vi "request OBW Measurement.vi"(8 "error in (no error)":errorcluster, 10 "Query Mode":T1, 11 "Keysight 9020A in":refnum<class "Keysight 9020A.lvclass">) -> (0 "error out":errorcluster, 2 "OBW Measurement Result Array":dbl[](array[numeric]), 3 "Keysight 9020A out":refnum<class "Keysight 9020A.lvclass">)   [LabVIEW 2023, in "Spectrum Analyzer.lvlib" / "Keysight 9020A.lvclass"]
uses:
  Keysight 9020A.lvclass
  TYPE DEFINITION/TYPE query Data Processing Type.ctl
  Keysight 9020A.lvclass/Keysight 9020A.ctl
  Spectrum Analyzer.lvlib
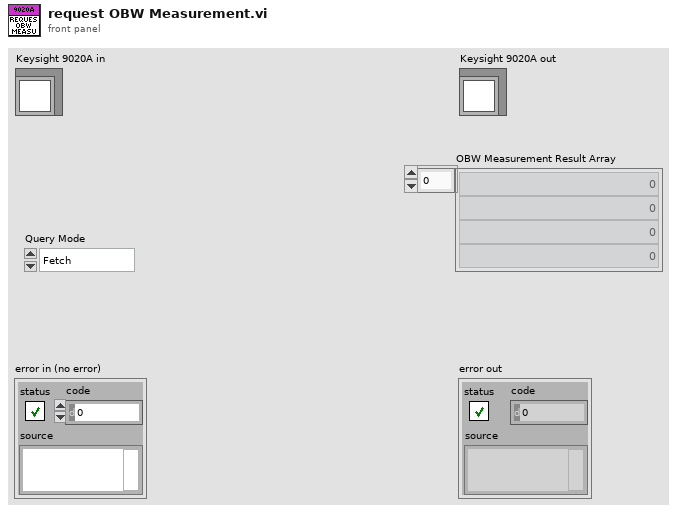
[diagram p1: front panel]
types:
  T1 = typedef "Spectrum Analyzer.lvlib/TYPE query Data Processing Type.ctl" = enum16{"Fetch", "Measure", "Read"}
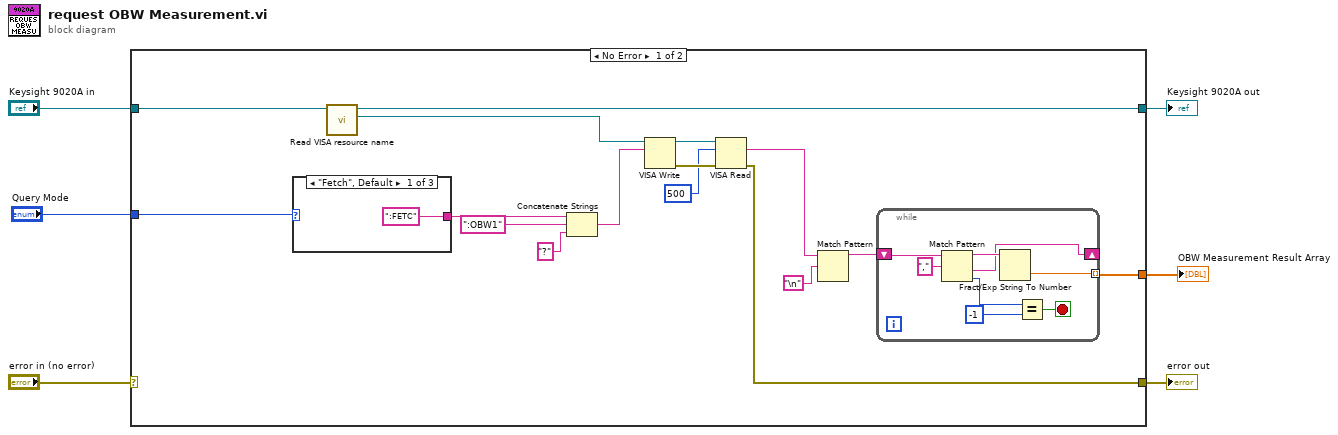
[diagram p0: block diagram]
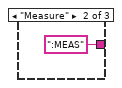
[diagram p2: hidden frame]
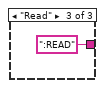
[diagram p3: hidden frame]
diagram:
  n1 = case shown="No Error" "error in (no error)" {
    selector: "error in (no error)" -> [_ w35]
    tunnel: [w8 w35] -> w5
    tunnel: [w18 w34] -> w3
    tunnel: "Keysight 9020A in" -> [w7 w34]
    tunnel: "Query Mode" -> [w19 _]
    tunnel: [w9 _] -> w1
    frame No Error {
      n2 = case shown="\"Fetch\", Default" w19 {
        tunnel: [":FETC" ":MEAS" ":READ"] -> w22
        frame "Fetch", Default {
        }
        frame "Measure" {
        }
        frame "Read" {
        }
      }
      n3 = call "Read VISA resource name.vi"("Keysight 9020A in"=w7) -> ("VISA resource name"=w11:refnum<visa-resource-name>, "Keysight 9020A out"=w18:refnum<class "Keysight 9020A.lvclass">)  [unwired: 8 in, 1 out]
      n4 = Concatenate Strings(w22, ":OBW1" ("string"), "?" ("string")) -> (w10:string)
      n5 = VISA Write(VISA resource name=w11, write buffer=w10) -> (VISA resource name out=w16:refnum<visa-resource-name>, error out=w17:errorcluster)  [unwired: 1 in, 1 out]
      n6 = VISA Read(VISA resource name=w16, byte count=u32 500, error in (no error)=w17) -> (read buffer=w14:string, error out=w8:errorcluster)  [unwired: 2 out]
      n7 = Match Pattern(string=w14, regular expression="\n") -> (before substring=w12:string)  [unwired: 1 in, 3 out]
      n8 = while {
        shift-right: [w26] -> _
        shift-left: w12 -> [w30]
        tunnel: [w27] -> w9 mode=indexing
        stop <- w23 stop-if-true
        n9 = Match Pattern(string=w30, regular expression=",") -> (before substring=w28:string, after substring=w26:string, offset past match=w25:i32)  [unwired: 1 in, 1 out]
        n10 = Fract/Exp String To Number(string=w28) -> (number=w27:dbl)  [unwired: 3 in, 1 out]
        n11 = Equal?(x=w25, y=-1) -> (x = y?=w23:bool)
      }
    }
    frame Error {
    }
  }
  "error out" <- w5
  "Keysight 9020A out" <- w3
  "OBW Measurement Result Array" <- w1
